vi "Write CIF Publisher Refnum.vi"(8 "error in (no error)":errorcluster, 10 "CIF Publisher Refnum":T1 {"refnum" format="%.0x"}, 11 "CIF_Iceoryx_PCAP_Universal in":refnum<class "CIF_Iceoryx_PCAP_Universal.lvclass">) -> (0 "error out":errorcluster, 3 "CIF_Iceoryx_PCAP_Universal out":refnum<class "CIF_Iceoryx_PCAP_Universal.lvclass">)   [LabVIEW 2021, in "CIF_Iceoryx_PCAP_Universal.lvclass"]
uses:
  CIF_Iceoryx_PCAP_Universal.lvclass
  <vilib>/CIF Foundation/CIF Iceoryx/Refnum/Typedef/CIF Publisher Refnum.ctl
  <vilib>/CIF Foundation/CIF Iceoryx/Iceoryx.lvlib
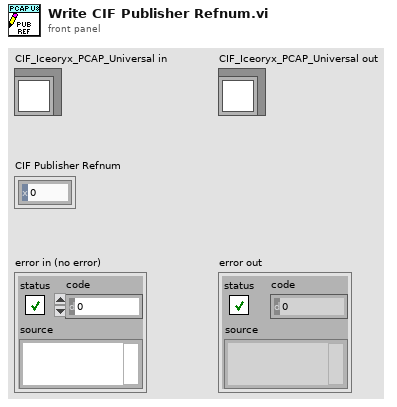
[diagram p1: front panel]
types:
  T1 = typedef "Iceoryx.lvlib/CIF Publisher Refnum.ctl" = cluster{"refnum":u64, "CIF Pub":enum8{"cifpub"}}
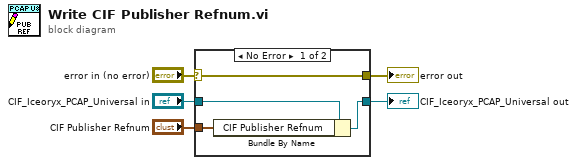
[diagram p0: block diagram]
diagram:
  n1 = case shown="No Error" "error in (no error)" {
    selector: "error in (no error)" -> [w9 w10]
    tunnel: [w9 w10] -> w4
    tunnel: [w7 w11] -> w2
    tunnel: "CIF_Iceoryx_PCAP_Universal in" -> [w8 w11]
    tunnel: "CIF Publisher Refnum" -> [w6 _]
    frame No Error {
      n2 = Bundle By Name(cluster=w8, "CIF Publisher Refnum"=w6) -> (w7:refnum<class "CIF_Iceoryx_PCAP_Universal.lvclass">)
    }
    frame Error {
    }
  }
  "error out" <- w4
  "CIF_Iceoryx_PCAP_Universal out" <- w2
